vi "pi_golden4.vi"() -> ()   [LabVIEW 2020]
panel:
  out "PI":dbl
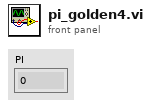
[diagram p1: front panel]
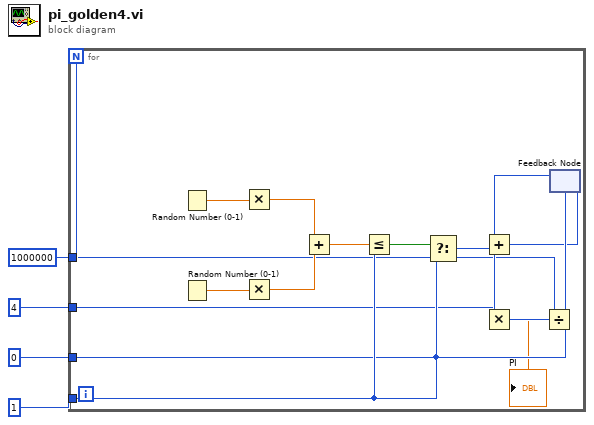
[diagram p0: block diagram]
diagram:
  w1 = 1000000 ("NConst")
  n1 = for "Loop1" {
    N: w1 -> [_]
    tunnel: 1 ("OneConst") -> [w19]
    tunnel: 0 ("ZeroConst") -> [w18]
    tunnel: 4 ("FourConst") -> [w8]
    tunnel: w1 -> [w6]
    n2 = Random Number (0-1) ("RN1")() -> (number: 0 to 1=w17:dbl)
    n3 = Random Number (0-1) ("RN2")() -> (number: 0 to 1=w16:dbl)
    n4 = Multiply ("SQX")(x=w17, y=w17) -> (x*y=w15:dbl)
    n5 = Multiply ("SQY")(x=w16, y=w16) -> (x*y=w14:dbl)
    n6 = Add ("R2")(x=w15, y=w14) -> (x+y=w13:dbl)
    n7 = Less Or Equal? ("LE1")(x=w13, y=w19) -> (x <= y?=w12:bool)
    n8 = Select ("SEL1")(t=w19, s=w12, f=w18) -> (s? t:f=w11:i32)
    n9 = feedback #1 ("FN1")(w18) -> (w10:i32)
    n10 = Add ("ACC")(x=w10, y=w11) -> (x+y=w9:i32)
    n11 = Multiply ("P")(x=w8, y=w9) -> (x*y=w7:i32)
    n12 = Divide ("DIV")(x=w7, y=w6) -> (x/y=→"PI":dbl)
    n13 = feedback-in #1(w9) -> ()
  }
